vi "RegisterActionEvent.vi"(8 "error in (no error)":errorcluster, 10 "Action":string, 11 "CONTROLLER in":refnum<class "CONTROLLER.lvclass">) -> (0 "error out":errorcluster, 3 "CONTROLLER out":refnum<class "CONTROLLER.lvclass">)   [LabVIEW 2013, in "CONTROLLER.lvclass"]
uses:
  CONTROLLER.lvclass
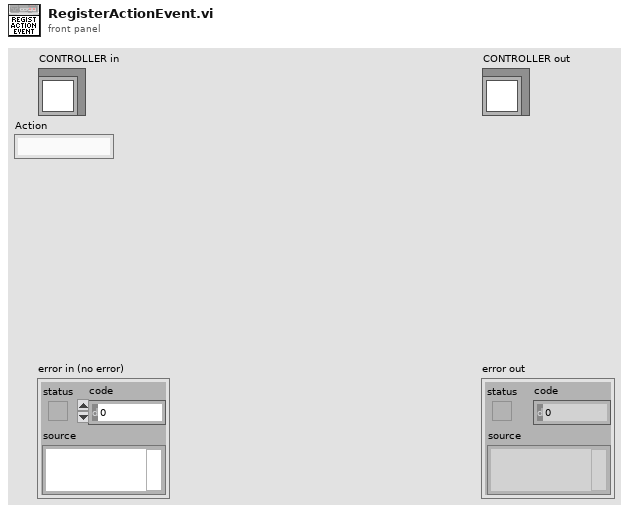
[diagram p1: front panel]
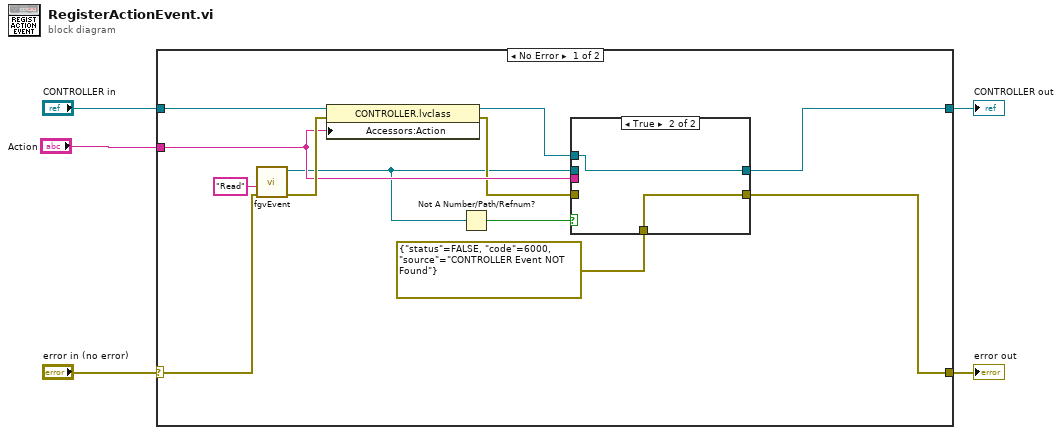
[diagram p0: block diagram]
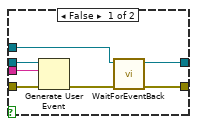
[diagram p2: hidden frame]
diagram:
  n1 = case shown="No Error" "error in (no error)" {
    selector: "error in (no error)" -> [w16 w28]
    tunnel: [w6 w28] -> w4
    tunnel: [w8 w27] -> w2
    tunnel: "CONTROLLER in" -> [w10 w27]
    tunnel: "Action" -> [w14 _]
    frame No Error {
      n2 = call "fgvEvent.vi"("error in (no error)"=w16, "Cmd"="Read") -> ("error out"=w15:errorcluster, "eventData Out"=w9:refnum<user-event>)  [unwired: 7 in, 1 out]
      n3 = property class="CONTROLLER.lvclass"(reference=w10, error in=w15, "Accessors:Action"=w14) -> (reference out=w7:refnum<class "CONTROLLER.lvclass">, error out=w13:errorcluster)
      n4 = Not A Number/Path/Refnum?(number/path/refnum=w9) -> (NaN/Path/Refnum?=w12:bool)
      n5 = case shown="True" w12 {
        tunnel: [w21 w26] -> w6
        tunnel: w14 -> [w24 _]
        tunnel: w13 -> [w23 _]
        tunnel: w9 -> [w22 _]
        tunnel: errorcluster {"status"=FALSE, "code"=6000, "source"="CONTROLLER Event NOT Found"} ("error out") -> [_ w26]
        tunnel: [w19 w25] -> w8
        tunnel: w7 -> [w18 w25]
        frame False {
          n6 = Generate User Event(user event=w22, event data cluster=w24, error in=w23) -> (error out=w20:errorcluster)  [unwired: 1 in, 1 out]
          n7 = call "WaitForEventBack.vi"("error in (no error)"=w20, "CONTROLLER in"=w18) -> ("error out"=w21:errorcluster, "CONTROLLER out"=w19:refnum<class "CONTROLLER.lvclass">)  [unwired: 8 in]
        }
        frame True {
        }
      }
    }
    frame Error {
    }
  }
  "error out" <- w4
  "CONTROLLER out" <- w2
